vi "~ct - Arg to DBL or CDB.vi"(7 "InstanceRef":T2, 8 "error in":bool, 9 "max args":i32=1, 10 "arg index":i32, 11 "args list":T3[](array[typedef])) -> (0 "CDB":cdb, 1 "2D CDB":cdb[][](array[numeric]), 2 "DBL":dbl, 3 "2D DBL":dbl[][](array[numeric]), 4 "error out":bool, 5 "category":T1(ring), 6 "arg type":T4=enum."DBL Number")   [LabVIEW 2021]
doc: "::: CalcExpress Toolkit :::\nCopyright (c) 2000-2026 Konstantin Shifershteyn. All rights reserved."
uses:
  cetypes.llb/CalcExpress Data Type.ctl
  cetypes.llb/CalcExpress Function Argument Info.ctl
  cetypes.llb/CalcExpress Instance RefNum.ctl
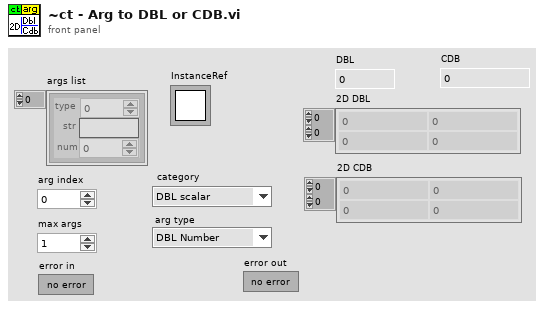
[diagram p1: front panel]
types:
  T1 = enum16{"DBL scalar", "CDB scalar", "DBL array", "CDB array", "ERROR"}
  T2 = typedef "CalcExpress Instance RefNum.ctl" = refnum<k1>
  T3 = typedef "CalcExpress Function Argument Info.ctl" = cluster{"type":u32, "str":string, "num":dbl}
  T4 = typedef "CalcExpress Data Type.ctl" = enum32{"String", "DBL Number", "identifier", "1D Array of DBL", "2D Array of DBL", "CDB Number", "1D Array of CDB", "2D Array of CDB", "1D Array of String", "2D Array of String", "Unknown data type"}
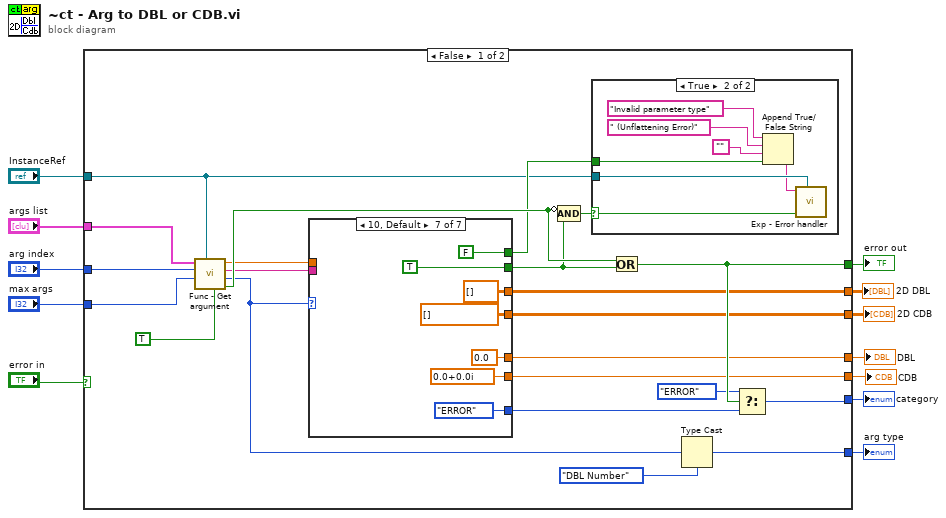
[diagram p0: block diagram]
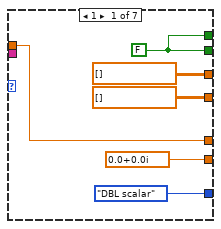
[diagram p3: hidden frame]
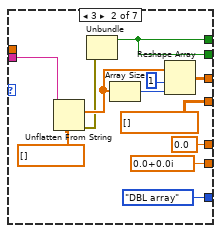
[diagram p4: hidden frame]
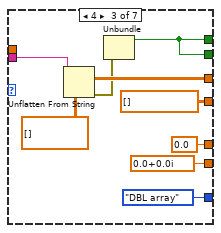
[diagram p5: hidden frame]
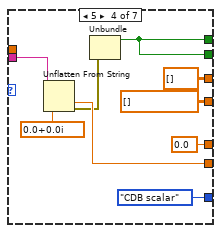
[diagram p6: hidden frame]
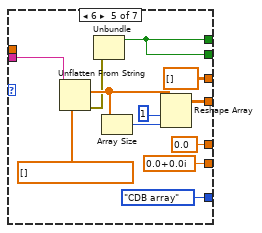
[diagram p7: hidden frame]
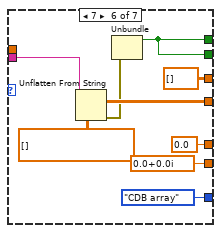
[diagram p8: hidden frame]
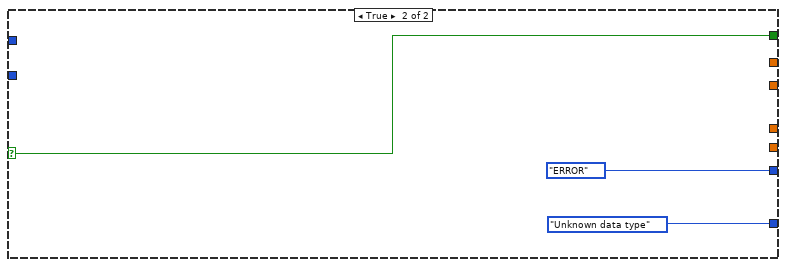
[diagram p9: hidden frame]
diagram:
  n1 = case shown="False" "error in" {
    selector: "error in" -> [_ w108]
    tunnel: [w27 w108] -> w11
    tunnel: [w26 T1."ERROR" ("category")] -> w10
    tunnel: "InstanceRef" -> [w23 _]
    tunnel: "args list" -> [w22 _]
    tunnel: "arg index" -> [w21 _]
    tunnel: "max args" -> [w20 _]
    tunnel: [w19 _] -> w5
    tunnel: [w18 _] -> w4
    tunnel: [w17 _] -> w3
    tunnel: [w16 _] -> w2
    tunnel: [w14 CalcExpress_Data_Type."Unknown data type" ("arg type")] -> w1
    frame False {
      n2 = call "Func - Get argument.vi"("ena NonNum? (F)"=TRUE ("ena complex? (F)"), "InstanceRef"=w23, "max arg num"=w20, "arg idx"=w21, "arg list"=w22) -> ("error out"=w34:bool, "type"=w15:u32, "str"=w32:string, "num"=w31:dbl)  [unwired: 1 in]
      n3 = case shown="10, Default" w15 {
        tunnel: [cdb[][] [] ("2D CDB") cdb[][] [] ("2D CDB") cdb[][] [] ("2D CDB") cdb[][] [] ("2D CDB") w87 w96 cdb[][] [] ("2D CDB")] -> w18
        tunnel: w32 -> [_ w59 w68 w76 w89 w98 _]
        tunnel: [w46 w55 w65 w74 w84 w94 TRUE ("err")] -> w33
        tunnel: [cdb 0.0+0.0i cdb 0.0+0.0i cdb 0.0+0.0i w75 cdb 0.0+0.0i cdb 0.0+0.0i cdb 0.0+0.0i] -> w16
        tunnel: w31 -> [w45 _ _ _ _ _ _]
        tunnel: [w46 w55 w65 w74 w84 w94 FALSE] -> w29
        tunnel: [dbl[][] [] ("2D CDB") w54 w64 dbl[][] [] ("2D CDB") dbl[][] [] ("2D CDB") dbl[][] [] ("2D CDB") dbl[][] [] ("2D CDB")] -> w19
        tunnel: [w45 0.0 ("num") 0.0 ("num") 0.0 ("num") 0.0 ("num") 0.0 ("num") 0.0 ("num")] -> w17
        tunnel: [T1."DBL scalar" ("category") T1."DBL array" ("category") T1."DBL array" ("category") T1."CDB scalar" ("category") T1."CDB array" ("category") T1."CDB array" ("category") T1."ERROR" ("category")] -> w28
        frame 1 {
          w46 = FALSE ("err")
        }
        frame 3 {
          n4 = Unflatten From String(type=dbl[] [], binary string=w59) -> (value=w57:dbl[], error out=w48:errorcluster)  [unwired: 3 in, 1 out]
          n5 = Unbundle(w48) -> ("status"=w55:bool)  [unwired: 2 out]
          n6 = Array Size(array=w57) -> (size(s)=w50:i32)
          n7 = Reshape Array(w57, 1, w50) -> (w54:dbl[][])
        }
        frame 4 {
          n8 = Unflatten From String(type=dbl[][] [], binary string=w68) -> (value=w64:dbl[][], error out=w60:errorcluster)  [unwired: 3 in, 1 out]
          n9 = Unbundle(w60) -> ("status"=w65:bool)  [unwired: 2 out]
        }
        frame 5 {
          n10 = Unflatten From String(type=cdb 0.0+0.0i, binary string=w76) -> (value=w75:cdb, error out=w69:errorcluster)  [unwired: 3 in, 1 out]
          n11 = Unbundle(w69) -> ("status"=w74:bool)  [unwired: 2 out]
        }
        frame 6 {
          n12 = Unflatten From String(type=cdb[] [], binary string=w89) -> (value=w85:cdb[], error out=w78:errorcluster)  [unwired: 3 in, 1 out]
          n13 = Unbundle(w78) -> ("status"=w84:bool)  [unwired: 2 out]
          n14 = Array Size(array=w85) -> (size(s)=w80:i32)
          n15 = Reshape Array(w85, 1, w80) -> (w87:cdb[][])
        }
        frame 7 {
          n16 = Unflatten From String(type=cdb[][] [], binary string=w98) -> (value=w96:cdb[][], error out=w90:errorcluster)  [unwired: 3 in, 1 out]
          n17 = Unbundle(w90) -> ("status"=w94:bool)  [unwired: 2 out]
        }
        frame 10, Default {
        }
      }
      n18 = Compound Arithmetic op=AND(invert w34, w33) -> (w30:bool)
      n19 = case shown="True" w30 {
        selector: w30 -> [_ w41]
        tunnel: w23 -> [_ w40]
        tunnel: w29 -> [_ w38]
        frame False {
        }
        frame True {
          n20 = Append True/False String(1:w38, 2:"", 3:" (Unflattening Error)" ("false string"), 4:"Invalid parameter type") -> (0:w39:string)
          n21 = call "Exp - Error handler.vi"("InstanceRef"=w40, "error in"=w41, "error message in"=w39) -> ()  [unwired: 6 in, 3 out]
        }
      }
      n22 = Or(x=w34, y=w33) -> (x .or. y?=w27:bool)
      n23 = Type Cast(type=CalcExpress_Data_Type."DBL Number" ("arg type"), x=w15) -> (*(type *) &x=w14:T4)
      n24 = Select(t=T1."ERROR", s=w27, f=w28) -> (s? t:f=w26:T1)
    }
    frame True {
    }
  }
  "error out" <- w11
  "category" <- w10
  "2D DBL" <- w5
  "2D CDB" <- w4
  "DBL" <- w3
  "CDB" <- w2
  "arg type" <- w1
